vi "Append Text Table to Report.vi"(0 "report in":refnum<class "ooCalc.lvclass">, 1 "column width (1)":dbl=1.0 format="%.2f", 2 "measurement system":u16(ring)=2 caption="measurement system for column width (Default)" items=["US", "Metric", "Default"], 3 "MS Office parameters":T2, 5 "column headers":string[](array[string]), 7 "row headers":string[](array[string]), 9 "text data":string[][](array[string]), 11 "error in (no error)":errorcluster, 13 "separate page?":bool, 14 "show grid lines":bool=TRUE) -> (4 "report out":refnum<class "ooCalc.lvclass">, 8 "range (wd) - start (xl)":T1, 10 "end (xl)":cluster{"row (xl) ":i32, "col (xl) ":i32}, 15 "error out":errorcluster)   [LabVIEW 2009, in "ooCalc.lvclass"]
doc: "Appends a 2D array to a report as a table with the given column width. You can use this polymorphic VI to append an array of strings or numbers. The data type you wire to the <B>text data</B> input determines the polymorphic instance to use."
uses:
  ooCalc.lvclass
  C:/Projets/LAVAG/OpenOfficeRGT/AODL/DLLs/AODL.dll
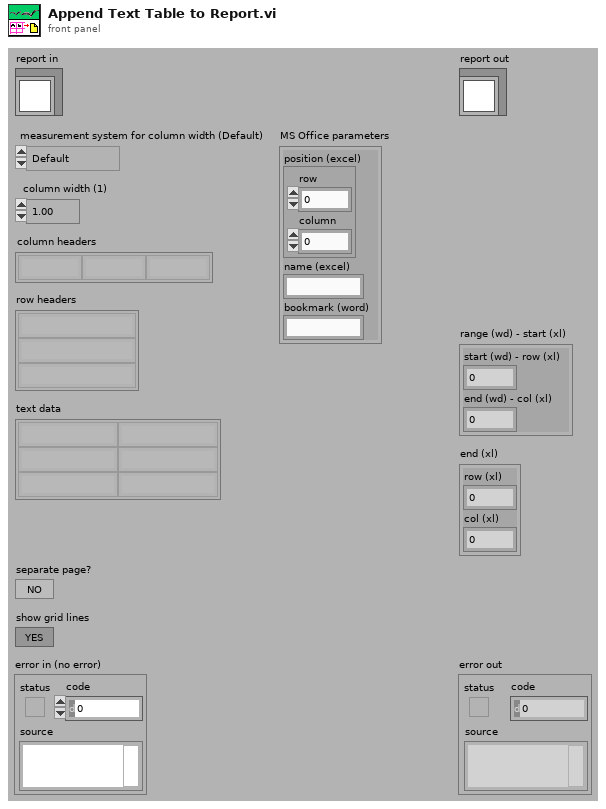
[diagram p1: front panel]
types:
  T1 = cluster{"start (wd) - row (xl) ":i32, "end (wd) - col (xl) ":i32}
  T2 = cluster{"position (excel)":cluster{"row":i32, "column":i32}, "name (excel)":string, "bookmark (word)":string}
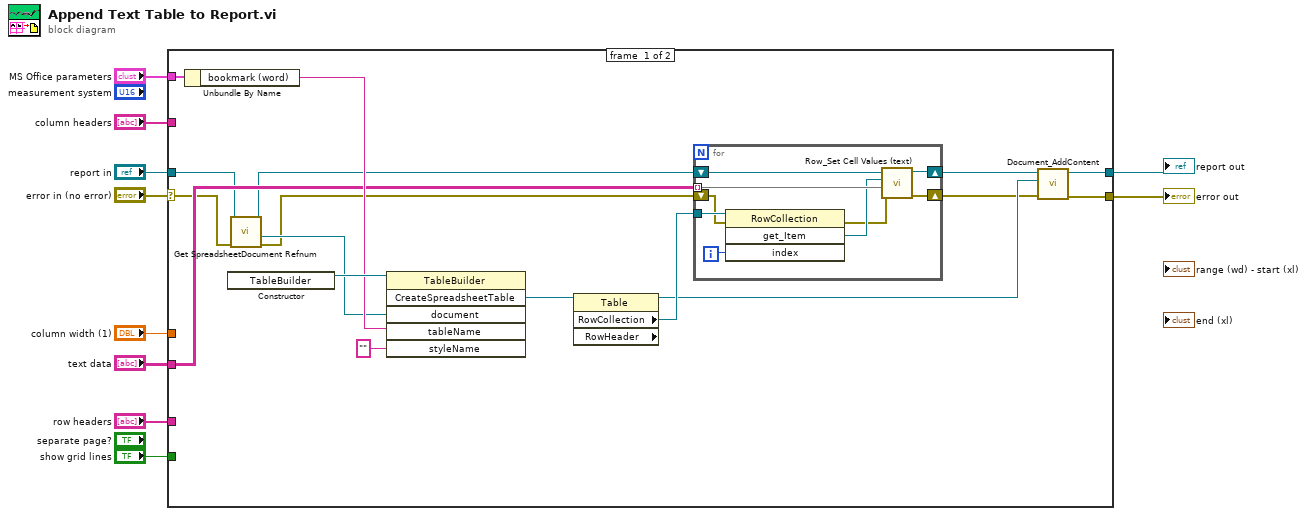
[diagram p0: block diagram]
diagram:
  n1 = case shown="No Error" "error in (no error)" {
    selector: "error in (no error)" -> [w12 w37]
    tunnel: [w21 w37] -> w9
    tunnel: "report in" -> [w15 w38]
    tunnel: [w22 w38] -> w7
    tunnel: "show grid lines" -> [_ _]
    tunnel: "text data" -> [w19 _]
    tunnel: "column width (1)" -> [_ _]
    tunnel: "MS Office parameters" -> [w26 _]
    tunnel: "column headers" -> [_ _]
    tunnel: "row headers" -> [_ _]
    frame #0 {
      n2 = Unbundle By Name(w26) -> ("bookmark (word)"=w25:string)
      n3 = constructor class="TableBuilder"() -> (reference out=w27:refnum<k24>)  [unwired: 3 in, 2 out]
      n4 = call-dynamic "Get SpreadsheetDocument Refnum.vi"("error in (no error)"=w12, "ooCalc in"=w15) -> ("error out"=w11:errorcluster, "SpreadsheetDocument"=w13:refnum<k24>, "ooCalc out"=w14:refnum<class "ooCalc.lvclass">)  [unwired: 7 in]
      n5 = invoke class="TableBuilder" method="CreateSpreadsheetTable"(reference=w27, "document"=w13, "tableName"=w25, "styleName"="") -> ("CreateSpreadsheetTable"=w23:refnum<k24>)  [unwired: 2 in, 5 out]
      n6 = property class="Table" props=["RowCollection", "RowHeader"](reference=w23) -> (reference out=w17:refnum<k24>, "RowCollection"=w18:refnum<k24>)  [unwired: 1 in, 2 out]
      n7 = for {
        shift-right: [w35] -> w20
        shift-left: w14 -> [w36]
        tunnel: w19 -> [w34] mode=indexing
        tunnel: w18 -> [w32]
        shift-right: [w29] -> w16
        shift-left: w11 -> [w28]
        i -> [w33]
        n8 = invoke class="RowCollection" method="get_Item"(reference=w32, error in=w28, "index"=w33) -> (error out=w30:errorcluster, "get_Item"=w31:refnum<k24>)  [unwired: 1 in, 2 out]
        n9 = call-dynamic "Row_Set Cell Values (text).vi"("error in (no error)"=w30, "text data (row)"=w34, "Row"=w31, "ooCalc in"=w36) -> ("error out"=w29:errorcluster, "ooCalc out"=w35:refnum<class "ooCalc.lvclass">)  [unwired: 6 in]
      }
      n10 = call-dynamic "Document_AddContent.vi"("error in (no error)"=w16, "Content"=w17, "ooCalc in"=w20) -> ("error out"=w21:errorcluster, "ooCalc out"=w22:refnum<class "ooCalc.lvclass">)  [unwired: 7 in]
    }
    frame #1 {
    }
  }
  "error out" <- w9
  "report out" <- w7
